vi "Call function.vi"(8 "error in":errorcluster, 10 "variant in":variant, 11 "connection ID":refnum<k5>) -> (0 "error out":errorcluster, 1 "data string out":string, 2 "JSON string out":string, 3 "connection ID out":refnum<k5>)   [LabVIEW 2020, in "LabVIEW-Python TCP Lib.lvlib"]
uses:
  LabVIEW-Python TCP Lib.lvlib
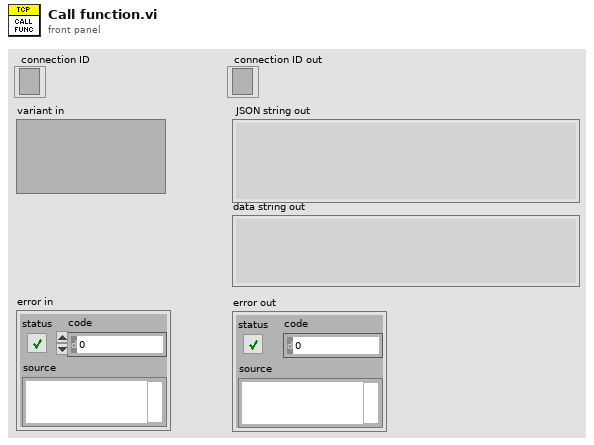
[diagram p1: front panel]
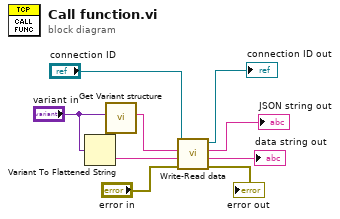
[diagram p0: block diagram]
diagram:
  n1 = Variant To Flattened String(Variant="variant in") -> (data string=w7:string)  [unwired: 1 out]
  n2 = call "Get Variant structure.vi"("variant in"="variant in") -> ("<JSON>"=w8:string)  [unwired: 10 in]
  n3 = call "Write-Read data.vi"("error in"="error in", "data string in"=w7, "JSON string in"=w8, "connection ID"="connection ID") -> ("error out"=→"error out":errorcluster, "data string out"=→"data string out":string, "JSON string out"=→"JSON string out":string, "connection ID out"=→"connection ID out":refnum<k5>)  [unwired: 4 in]
